vi "SMS Image Preview.vi"(7 "Calling VI Ref":refnum<vi>) -> ()   [LabVIEW 2021]
uses:
  <vilib>/Utility/miscctls.llb/LVPointTypeDef.ctl
  Hardware Configuration/Hardware Configuration Controls/Device Function.ctl
  SMS Image Preview Type Defs/SMS Image Preview Notifier Type.ctl
  SMS Image Preview Type Defs/SMS Image Preview Actions.ctl
  <vilib>/vision/Image Controls.llb/IMAQ Image.ctl
  Device Library/Cameras/Hamamatsu/Orca Flash/Orca Flash Controls/Orca Flash Actions.ctl
  Hardware Configuration/Hardware Configuration Controls/Device Type.ctl
  Device Library/FPGA/FPGA Controls/FPGA Action.ctl
  Device Library/Cameras/Camera Controls/Camera IMAQ Key Info.ctl
  Device Library/Lasers/Laser Controls/Laser Actions.ctl
  Device Library/Lasers/Laser Controls/Laser Settings.ctl
  Device Library/Lasers/Laser Controls/Laser Parameters.ctl
  <vilib>/Analysis/baseanly.llb/Mean (DBL).vi
  <vilib>/vision/NI_Vision_Development_Module.lvlib
  <vilib>/Analysis/NI_AALBase.lvlib
panel:
  in  "Laser":u16(ring) items=["405", "488"]
  in  "YOffset":i32=-1
  in  "XOffset":i32=1
  in  "Angle (degrees)":sgl format="%.2f"
  out "Current Emitter No.":u16
  in  "Duration":u32 max=65535 step=1
  in  "P Const.":dbl=0.5
  in  "Target Emitter No.":u16=3
  in  "Lock Density":bool
  in  "Average Frame No.":i32=2
  in  "Edge Size":i32=12
  in  "Use Quadrant":bool
  in  "Reset Plot":bool
  out "Blink No. vs. Time":cluster{dbl[], u16[]}(graph)
  in  "Accumulate":bool
  in  "Blink Sensitivity":sgl=10.0
  in  "Image Display":bool
  in  "SMS Preview":bool
  in  "Camera ROI":bool
  in  "Camera":i32(ring) items=["Hamamatsu-Camera-Primary-0"]
  in  "Quit":bool
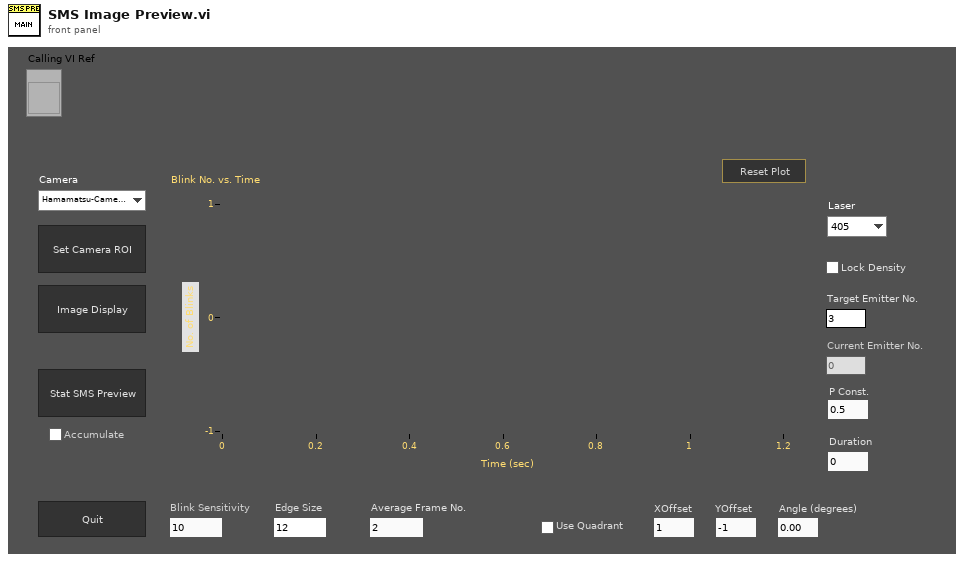
[diagram p1: front panel]
types:
  T1 = typedef "Device Function.ctl" = enum16{"Primary", "Secondary", "Overview", "Wide Field Drift Correction", "642 nm Excitation", "560 nm Excitation", "940 nm Excitation", "546 nm Excitation", "488 nm Excitation", "405 nm Excitation", "Objective Drift Correction", "4Pi Focus Lock", "4Pi Objective Lock", "Objective XY", "Objective Z", "Sample XY", "Sample Coarse Z", "Sample Z", "4Pi Lower", "4Pi Upper", "Em Small", "Em Large", "Ex Small", "Ex Large", "Mojo", "Adj Cavity", "Line Scanning", "Alert"}
  T2 = typedef "Image Type" = u32
  T3 = typedef "FPGA Action.ctl" = enum16{"Set Laser Mode", "Set Sequence", "Set Duration", "Write Check", "Idle", "Quit"}
  T4 = typedef "Device Type.ctl" = enum16{"AOTF", "Camera", "Deformable Mirror", "Laser", "Flip Mirror", "Shutter", "Stage", "Waveform", "FPGA", "Filter Wheel", "Email"}
  T5 = enum8{"Enabled", "Disabled", "Disabled and Grayed Out"}
  T6 = typedef "Orca Flash Actions.ctl" = enum16{"IDLE", "PREVIEW", "RECORD", "Send Trigger", "SOFT TRIGGER", "Record Settings", "SETPARAM", "GETPARAM", "SETROI", "GETROI", "PROGRESSIVE MODE", "AREA MODE", "STATUS", "QUIT"}
  T7 = typedef "SMS Image Preview Actions.ctl" = enum16{"Idle", "Start SMS Preview", "Get Image", "Get Quad", "Sum Quad", "Convolve and Threshold", "Subtract > Dilate", "And Image", "Remove Edge", "Update Plot", "Update Duration", "Abort", "Exit Loop", "Quit"}
  T8 = typedef "SMS Image Preview Notifier Type.ctl" = cluster{"Action":T7, "Camera Notifier Name":string, "Camera Image (U16)":T9, "Camera ROI":cluster{"Global Rectangle":i32[], "Contours":cluster{"Contour Type":u32, "ROI Type":u32, "Points":i32[]}[]}, "SMS Preview (U16)":T9, "Camera ROI (U16)":T9, "Threshold (U16)":T9, "Subtracted > Dilated (U16)":T9, "And Image (U16)":T9, "Camera ROI (SGL)":T9, "Conv 5 x 5 (SGL)":T9, "Conv 11 x 11 (SGL)":T9, "Subtracted (SGL)":T9, "Dilated (SGL)":T9, "Subtracted > Dilated (SGL)":T9, "Ones 5 x 5":sgl[][], "Ones 11 x 11":sgl[][], "Ones 7 x 7":i32[][], "Quads":T9[], "Edge Removed (U16)":T9, "Laser Notifier Name":string, "FPGA Notifier Name":string, "Duration":u32, "Quad 3 TM":T9}
  T9 = typedef "IMAQ Image.ctl" = refnum<image>
  T10 = enum16{"Always On", "Always Off", "Off While Running"}
  T11 = typedef "LVPointTypeDef.ctl" = cluster{"Horizontal":i16, "Vertical":i16}
  T12 = typedef "Camera IMAQ Key Info.ctl" = cluster{"Frame":u32, "Sensor Height":i32, "Sensor Width":i32, "ROI Height":i32, "ROI Width":i32, "ROI Enable?":bool, "Bit per Pixel":u8}
  T13 = enum32{"Average", "Min", "Max", "Clear  if < ", "Clear  if < or =", "Clear  if =", "Clear  if > or =", "Clear  if >"}
  T14 = enum32{"AutoM", "Close", "Dilate", "Erode", "Gradient", "Gradient in", "Gradient out", "HitMiss", "Open", "PClose", "POpen", "Thick", "Thin"}
  T15 = enum32{"Invalid", "Standard", "Closed", "Hidden", "Minimized", "Maximized"}
  T16 = cluster{"Global Rectangle":i32[], "Contours":cluster{"Contour Type":u32, "ROI Type":u32, "Points":i32[]}[]}
  T17 = typedef "Laser Parameters.ctl" = enum16{"Wavelength (nm)", "Pulsing?", "Rep. Rate", "External Control", "Enable Fine", "Fine A", "Fine B", "Channel No."}
  T18 = typedef "Laser Settings.ctl" = cluster{"Laser Parameters":T17, "Value":dbl}
  T19 = typedef "Laser Actions.ctl" = enum16{"Error Check", "Set On/Off", "Set Power", "Set Parameter", "Get Power", "Get Status", "Get Parameter", "Quit"}
  T20 = cluster{"histogram":u32[], "Minimal Value":sgl, "Maximal Value":sgl, "Starting Value":sgl, "Interval Width":sgl, "Mean Value":sgl, "Standard  Variation":sgl, "Area (pixels)":i32}
  T21 = typedef "LVRectTypeDef.ctl" = cluster{"Left":i16, "Top":i16, "Right":i16, "Bottom":i16}
  T22 = typedef "LVBoundsTypeDef.ctl" = cluster{"Width":u32, "Height":u32}
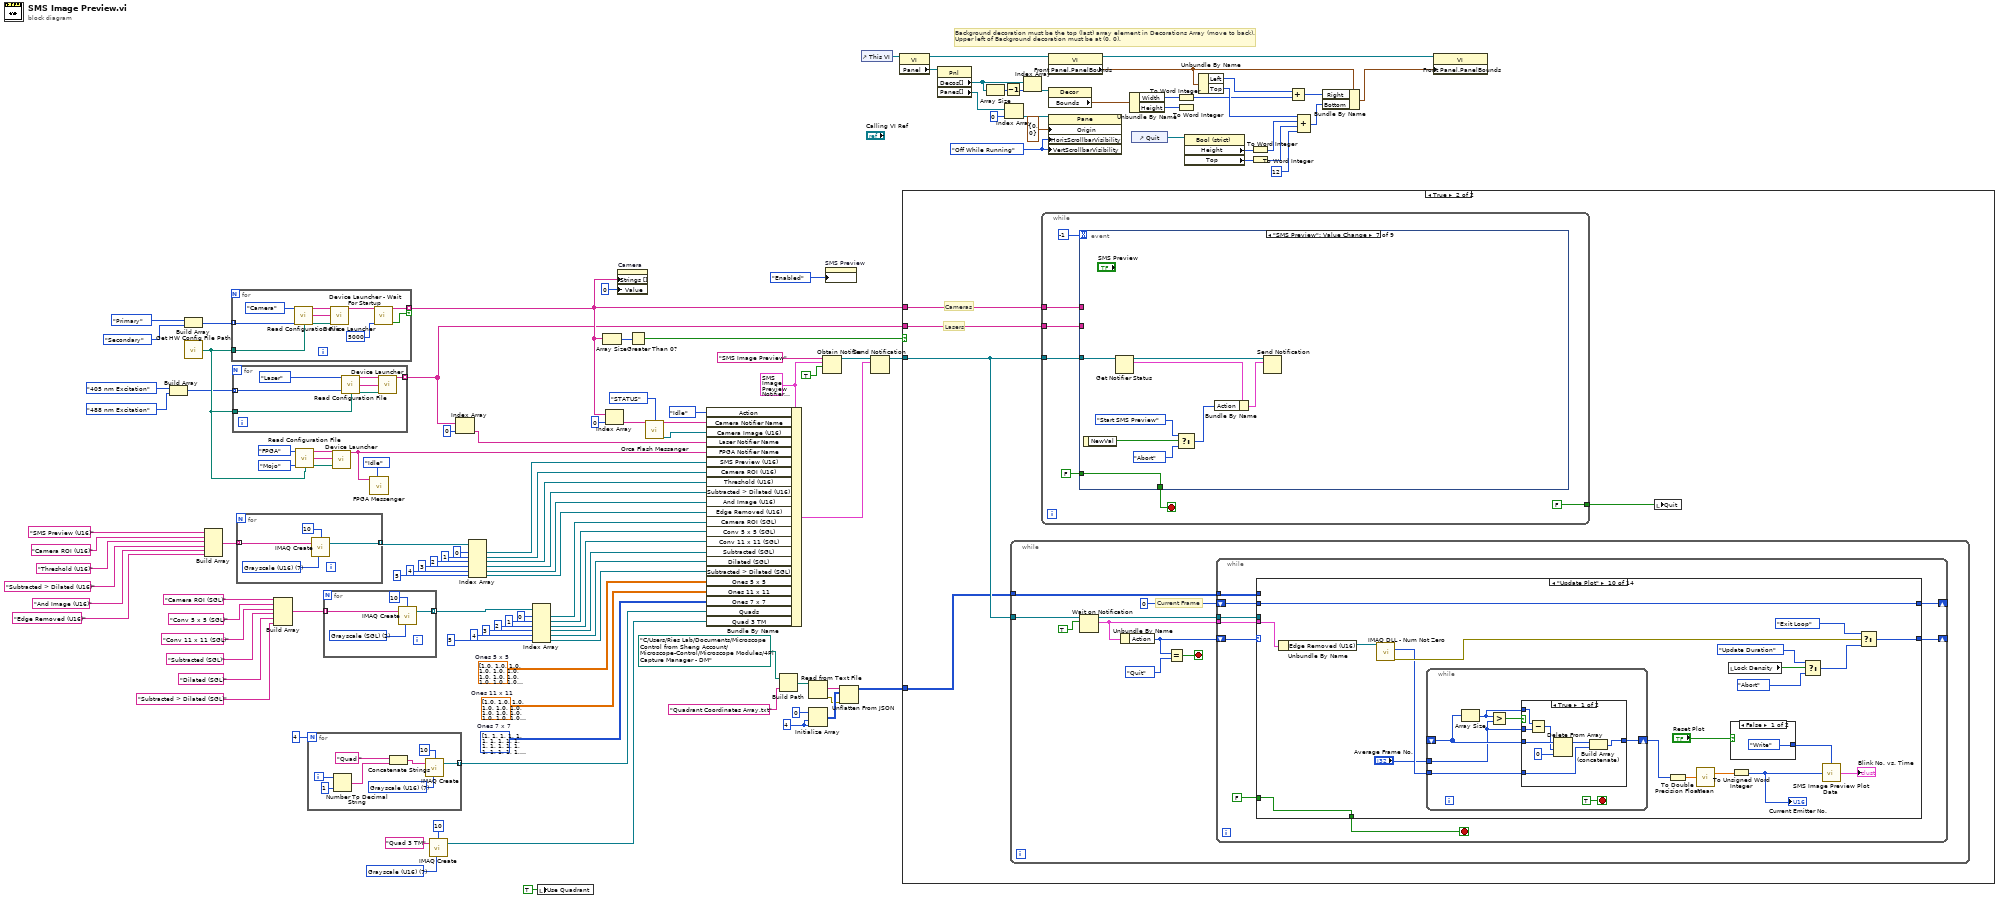
[diagram p0: block diagram]
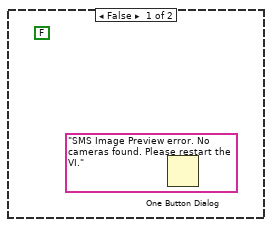
[diagram p2: hidden frame]
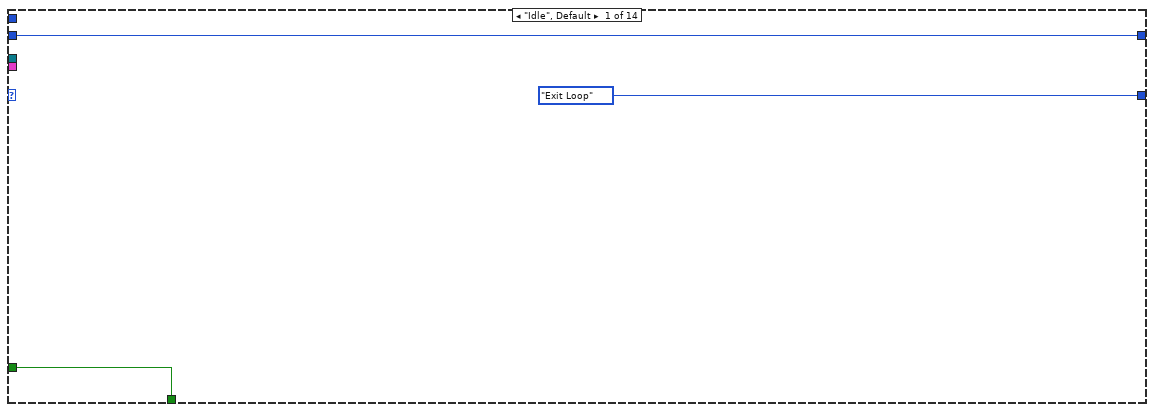
[diagram p3: hidden frame]
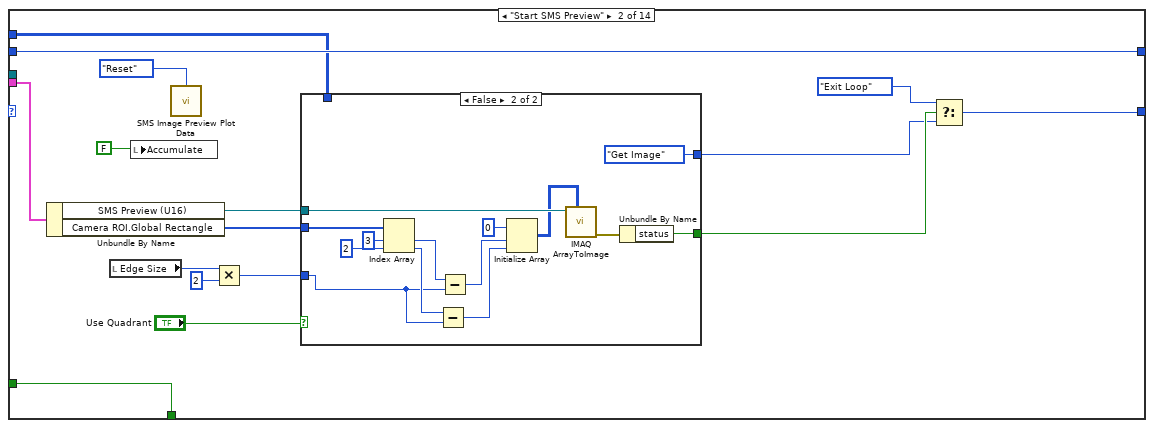
[diagram p4: hidden frame]
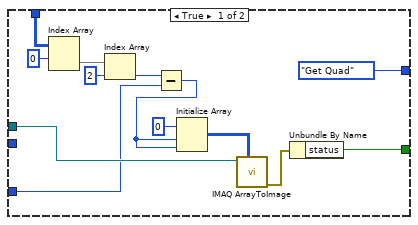
[diagram p5: hidden frame]
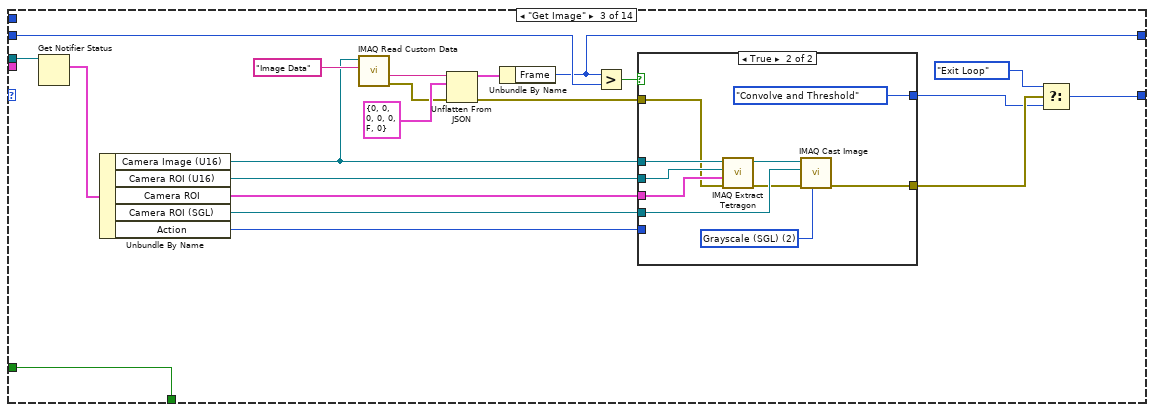
[diagram p6: hidden frame]
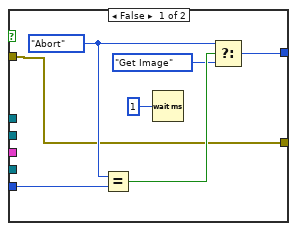
[diagram p7: hidden frame]
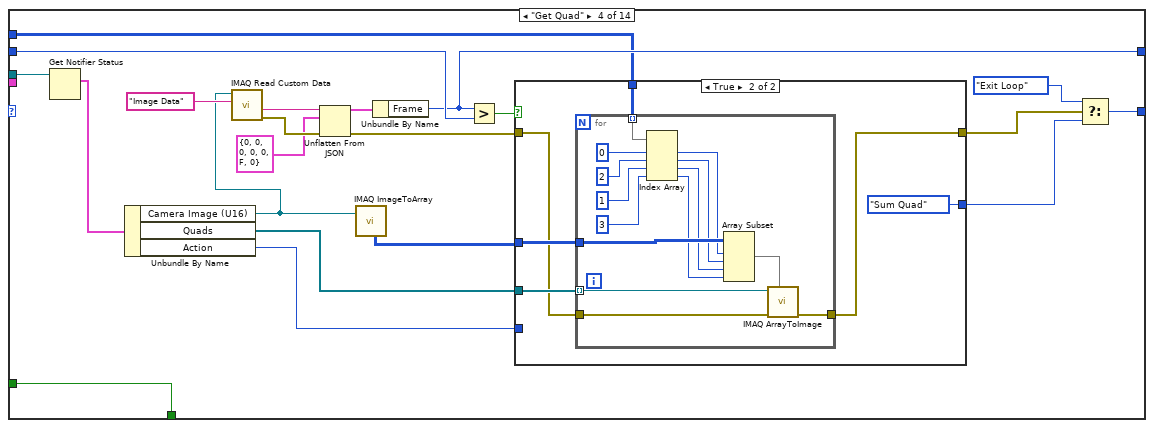
[diagram p8: hidden frame]
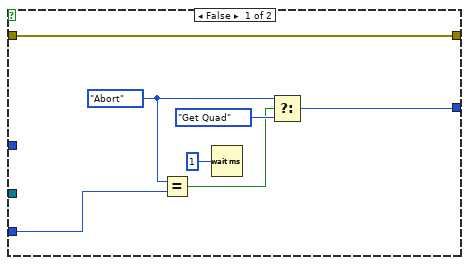
[diagram p9: hidden frame]
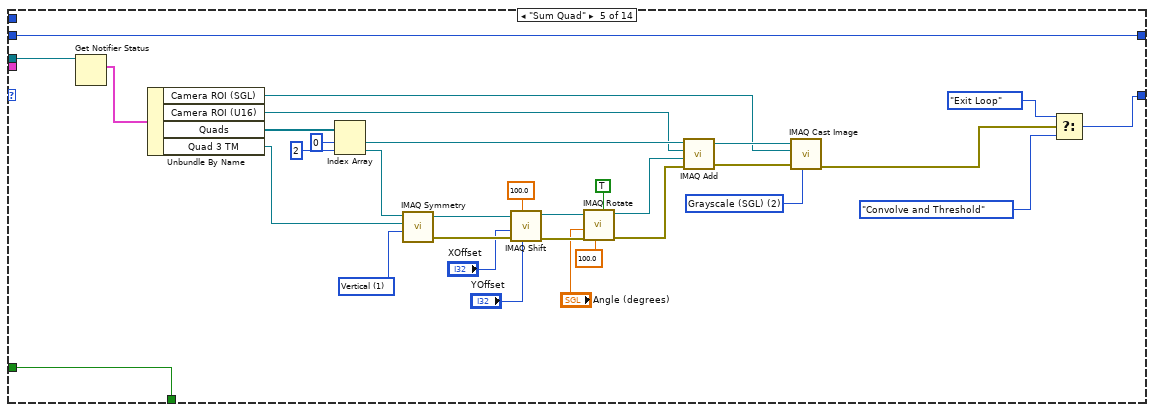
[diagram p10: hidden frame]
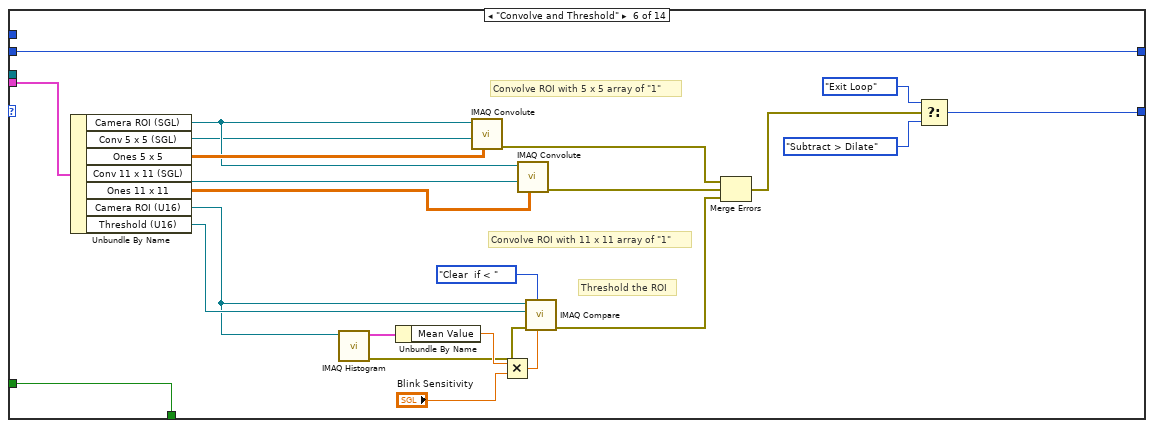
[diagram p11: hidden frame]
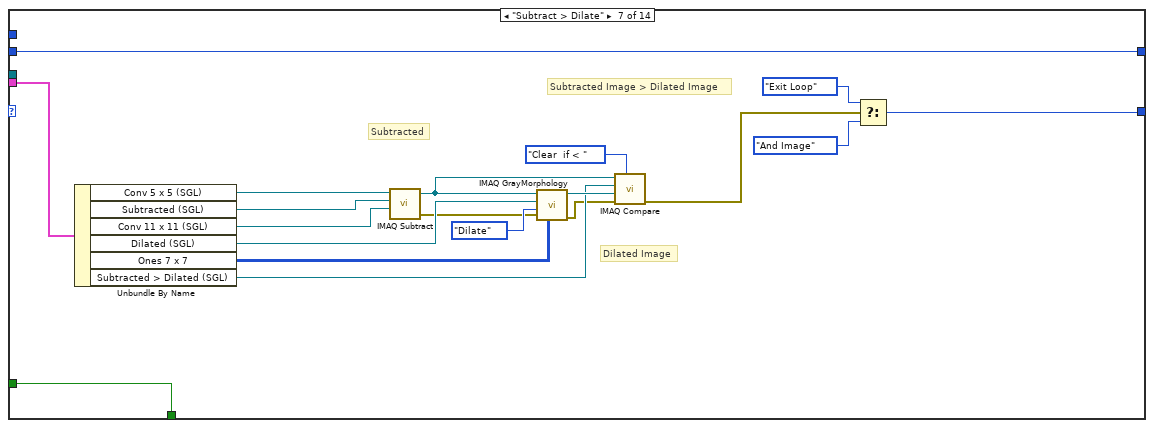
[diagram p12: hidden frame]
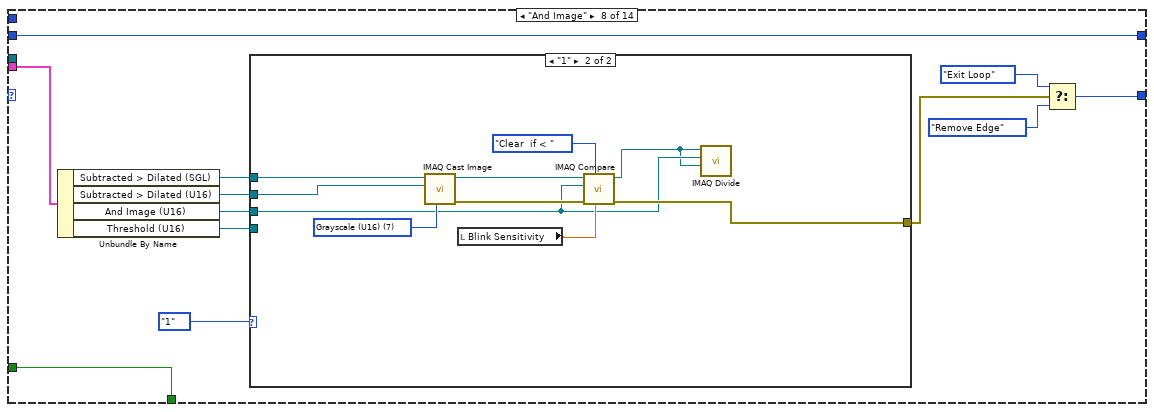
[diagram p13: hidden frame]
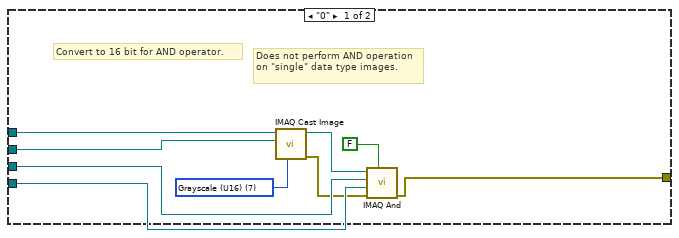
[diagram p14: hidden frame]
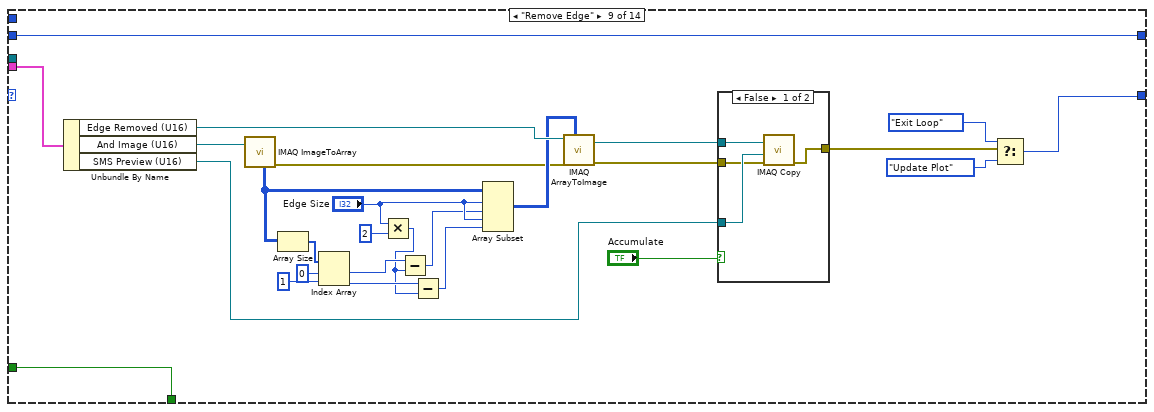
[diagram p15: hidden frame]
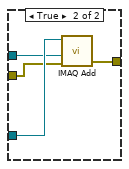
[diagram p16: hidden frame]
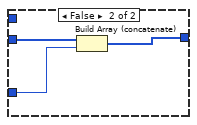
[diagram p17: hidden frame]
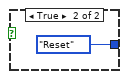
[diagram p18: hidden frame]
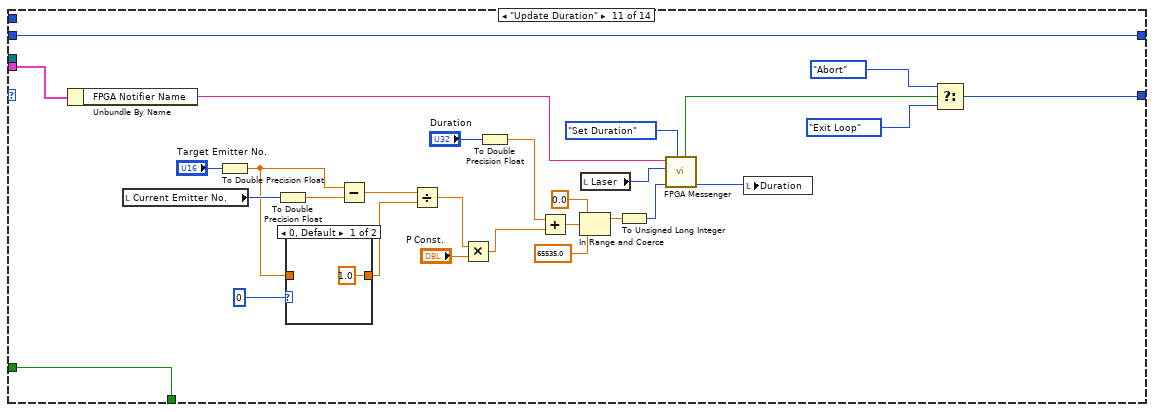
[diagram p19: hidden frame]
diagram:
  w12 = T2 7 items=["Grayscale (U8)", "Grayscale (I16)", "Grayscale (SGL)", "Complex (CSG)", "RGB (U32)", "HSL (U32)", "RGB (U64)", "Grayscale (U16)"] ("Image Type")
  w27 = 4 ("dimension size")
  w38 = i32[][] [[1, 1, 1, 1, 1, 1, 1], [1, 1, 1, 1, 1, 1, 1], [1, 1, 1, 1, 1, 1, 1], [1, 1, 1, 1, 1, 1, 1], [1, 1, 1, 1, 1, 1, 1], [1, 1, 1, 1, 1, 1, 1], [1, 1, 1, 1, 1, 1, 1]]  # Ones 7 x 7
  w39 = sgl[][] [[1.0, 1.0, 1.0, 1.0, 1.0, 1.0, 1.0, 1.0, 1.0, 1.0, 1.0], [1.0, 1.0, 1.0, 1.0, 1.0, 1.0, 1.0, 1.0, 1.0, 1.0, 1.0], [1.0, 1.0, 1.0, 1.0, 1.0, 1.0, 1.0, 1.0, 1.0, 1.0, 1.0], [1.0, 1.0, 1.0, 1.0, 1.0, 1.0, 1.0, 1.0, 1.0, 1.0, 1.0], [1.0, 1.0, 1.0, 1.0, 1.0, 1.0, 1.0, 1.0, 1.0, 1.0, 1.0], [1.0, 1.0, 1.0, 1.0, 1.0, 1.0, 1.0, 1.0, 1.0, 1.0, 1.0], [1.0, 1.0, 1.0, 1.0, 1.0, 1.0, 1.0, 1.0, 1.0, 1.0, 1.0], [1.0, 1.0, 1.0, 1.0, 1.0, 1.0, 1.0, 1.0, 1.0, 1.0, 1.0], [1.0, 1.0, 1.0, 1.0, 1.0, 1.0, 1.0, 1.0, 1.0, 1.0, 1.0], [1.0, 1.0, 1.0, 1.0, 1.0, 1.0, 1.0, 1.0, 1.0, 1.0, 1.0], [1.0, 1.0, 1.0, 1.0, 1.0, 1.0, 1.0, 1.0, 1.0, 1.0, 1.0]]  # Ones 11 x 11
  w40 = sgl[][] [[1.0, 1.0, 1.0, 1.0, 1.0], [1.0, 1.0, 1.0, 1.0, 1.0], [1.0, 1.0, 1.0, 1.0, 1.0], [1.0, 1.0, 1.0, 1.0, 1.0], [1.0, 1.0, 1.0, 1.0, 1.0]]  # Ones 5 x 5
  w35 = T8 {"Action"=enum."Idle", "Camera Notifier Name"="", "Camera Image (U16)"=refnum, "Camera ROI"={"Global Rectangle"=[], "Contours"=[]}, "SMS Preview (U16)"=refnum, "Camera ROI (U16)"=refnum, "Threshold (U16)"=refnum, "Subtracted > Dilated (U16)"=refnum, "And Image (U16)"=refnum, "Camera ROI (SGL)"=refnum, "Conv 5 x 5 (SGL)"=refnum, "Conv 11 x 11 (SGL)"=refnum, "Subtracted (SGL)"=refnum, "Dilated (SGL)"=refnum, "Subtracted > Dilated (SGL)"=refnum, "Ones 5 x 5"=[], "Ones 11 x 11"=[], "Ones 7 x 7"=[], "Quads"=[], "Edge Removed (U16)"=refnum, "Laser Notifier Name"="", "FPGA Notifier Name"="", "Duration"=0, "Quad 3 TM"=refnum} ("SMS Image Preview Notifier Type")
  w105 = T10."Off While Running" ("Vertical Scrollbar Visibility")
  # "Background decoration must be the top (last) array element in Decorations Array (move to back).\nUpper left of Background decoration must be at (0, 0)."
  n1 = Build Array(Device_Function."405 nm Excitation" ("Device Function"), Device_Function."488 nm Excitation" ("Device Function")) -> (w5:T1[])
  n2 = Build Array(Device_Function."Primary" ("Device Function"), Device_Function."Secondary" ("Device Function")) -> (w91:T1[])
  n3 = call "Get HW Config File Path.vi"() -> ("File Path"=w15:path)  [unwired: 14 in, 1 out]
  n4 = Build Array("SMS Preview (U16)" ("Image Name"), "Camera ROI (U16)" ("Image Name"), "Threshold (U16)" ("Image Name"), "Subtracted > Dilated (U16)" ("Image Name"), "And Image (U16)" ("Image Name"), "Edge Removed (U16)" ("element")) -> (w50:string[])
  n5 = for {
    tunnel: w91 -> [w128] mode=indexing
    tunnel: w15 -> [w127]
    tunnel: [w125] -> w81 mode=indexing if=w124
    n6 = call "Read Configuration File.vi"("Device Type"=Device_Type."Camera", "Device Function"=w128, "Config File Path"=w127) -> ("Unique Notifier Name"=w130:string, "Device Ports/IDs/Channels"=w132:string[], "Device Engine Path"=w131:path)  [unwired: 9 in, 1 out]
    n7 = call "Device Launcher.vi"("Notifier Name"=w130, "Device Ports/IDs/Channels"=w132, "Device Engine Path"=w131) -> ("Notifier Name"=w126:string)  [unwired: 11 in, 1 out]
    n8 = call "Device Launcher - Wait For Startup.vi"("Notifier Name"=w126, "Wait Time (ms)"=5000) -> ("Notifier Name (Dup)"=w125:string, "Running?"=w124:bool)  [unwired: 12 in]
  }
  n9 = for {
    tunnel: [w135] -> w2 mode=indexing
    tunnel: w15 -> [w134]
    tunnel: w5 -> [w133] mode=indexing
    n10 = call "Read Configuration File.vi"("Device Type"=Device_Type."Laser", "Device Function"=w133, "Config File Path"=w134) -> ("Unique Notifier Name"=w138:string, "Device Ports/IDs/Channels"=w137:string[], "Device Engine Path"=w136:path)  [unwired: 9 in, 1 out]
    n11 = call "Device Launcher.vi"("Notifier Name"=w138, "Device Ports/IDs/Channels"=w137, "Device Engine Path"=w136) -> ("Notifier Name"=w135:string)  [unwired: 11 in, 1 out]
  }
  n12 = for {
    tunnel: w50 -> [w141] mode=indexing
    tunnel: [w140] -> w51 mode=indexing
    w142 = T2 7 items=["Grayscale (U8)", "Grayscale (I16)", "Grayscale (SGL)", "Complex (CSG)", "RGB (U32)", "HSL (U32)", "RGB (U64)", "Grayscale (U16)"] ("Image Type")
    n13 = call "IMAQ Create"("Border Size"=10, "Image Name"=w141, "Image Type"=w142) -> ("New Image"=w140:T9)  [unwired: 2 in, 1 out]
  }
  n14 = Build Array("Camera ROI (SGL)" ("Image Name"), "Conv 5 x 5 (SGL)" ("Image Name"), "Conv 11 x 11 (SGL)" ("Image Name"), "Subtracted (SGL)" ("Image Name"), "Dilated (SGL)" ("Image Name"), "Subtracted > Dilated (SGL)" ("Image Name")) -> (w70:string[])
  n15 = call "Read Configuration File.vi"("Device Type"=Device_Type."FPGA", "Device Function"=Device_Function."Mojo", "Config File Path"=w15) -> ("Unique Notifier Name"=w18:string, "Device Ports/IDs/Channels"=w17:string[], "Device Engine Path"=w16:path)  [unwired: 9 in, 1 out]
  n16 = for {
    N: 4 -> [_]
    tunnel: [w149] -> w34 mode=indexing
    i -> [w148]
    w151 = T2 7 items=["Grayscale (U8)", "Grayscale (I16)", "Grayscale (SGL)", "Complex (CSG)", "RGB (U32)", "HSL (U32)", "RGB (U64)", "Grayscale (U16)"] ("Image Type")
    n17 = Number To Decimal String(number=w148, width (-)=i16 1) -> (decimal integer string=w145:string)
    n18 = Concatenate Strings("Quad " ("Image Name"), w145) -> (w144:string)
    n19 = call "IMAQ Create"("Border Size"=10, "Image Name"=w144, "Image Type"=w151) -> ("New Image"=w149:T9)  [unwired: 2 in, 1 out]
  }
  n20 = for {
    tunnel: w70 -> [w153] mode=indexing
    tunnel: [w152] -> w69 mode=indexing
    w154 = T2 2 items=["Grayscale (U8)", "Grayscale (I16)", "Grayscale (SGL)", "Complex (CSG)", "RGB (U32)", "HSL (U32)", "RGB (U64)", "Grayscale (U16)"] ("Image Type")
    n21 = call "IMAQ Create"("Border Size"=10, "Image Name"=w153, "Image Type"=w154) -> ("New Image"=w152:T9)  [unwired: 2 in, 1 out]
  }
  n22 = call "Device Launcher.vi"("Notifier Name"=w18, "Device Ports/IDs/Channels"=w17, "Device Engine Path"=w16) -> ("Notifier Name"=w14:string)  [unwired: 11 in, 1 out]
  n23 = call "FPGA Messenger.vi"("FPGA Action"=FPGA_Action."Idle", "Notifier Name"=w14) -> ()  [unwired: 4 in, 6 out]
  n24 = call "IMAQ Create"("Border Size"=10, "Image Name"="Quad 3 TM", "Image Type"=w12) -> ("New Image"=w9:T9)  [unwired: 2 in, 1 out]
  n25 = Index Array(array=w2, index=0) -> (element=w3:string)
  n26 = Index Array(array=w51, index #1=0 ("index"), index #2=1 ("index"), index #3=2 ("index"), index #4=3 ("index"), index #5=4 ("index"), index #6=5 ("index")) -> (element #1=w49:T9, element #2=w48:T9, element #3=w47:T9, element #4=w23:T9, element #5=w22:T9, element #6=w21:T9)
  n27 = Index Array(array=w69, index #1=0 ("index"), index #2=1 ("index"), index #3=2 ("index"), index #4=3 ("index"), index #5=4 ("index"), index #6=5 ("index")) -> (element #1=w46:T9, element #2=w45:T9, element #3=w44:T9, element #4=w43:T9, element #5=w42:T9, element #6=w41:T9)
  n28 = local write "Use Quadrant"(TRUE ("Use Quadrant")) -> ()
  n29 = Array Size(array=w81) -> (size(s)=w90:i32)
  n30 = Index Array(array=w81, index=0) -> (element=w79:string)
  n31 = property on="Camera" class="Ring (strict)"("Strings []"=w81, "Value"=0) -> ()  [unwired: 2 in, 2 out]
  n32 = Greater Than 0?(x=w90) -> (x > 0?=w89:bool)
  n33 = call "Orca Flash Messanger.vi"("Notifier Name"=w79, "Camera Actions"=Orca_Flash_Actions."STATUS") -> ("Notifier Name Dup"=w78:string, "Image Ref"=w76:T9)  [unwired: 9 in, 3 out]
  n34 = Bundle By Name(cluster=w35, "Action"=SMS_Image_Preview_Actions."Idle", "Camera Notifier Name"=w78, "Camera Image (U16)"=w76, "Laser Notifier Name"=w3, "FPGA Notifier Name"=w14, "SMS Preview (U16)"=w49, "Camera ROI (U16)"=w48, "Threshold (U16)"=w47, "Subtracted > Dilated (U16)"=w23, "And Image (U16)"=w22, "Edge Removed (U16)"=w21, "Camera ROI (SGL)"=w46, "Conv 5 x 5 (SGL)"=w45, "Conv 11 x 11 (SGL)"=w44, "Subtracted (SGL)"=w43, "Dilated (SGL)"=w42, "Subtracted > Dilated (SGL)"=w41, "Ones 5 x 5"=w40, "Ones 11 x 11"=w39, "Ones 7 x 7"=w38, "Quads"=w34, "Quad 3 TM"=w9) -> (w82:T8)
  n35 = Build Path(base path=path "C:/Users/Ries Lab/Documents/Microscope Control from Sheng Account/Microscope-Control/Microscope Modules/4Pi Capture Manager - DM" ("path"), name or relative path="Quadrant Coordinates Array.txt") -> (appended path=w30:path)
  n36 = Read from Text File(file (use dialog)=w30) -> (text=w29:string, error out=w28:errorcluster)  [unwired: 3 in, 2 out]
  n37 = Initialize Array(0 ("element"), w27, w27) -> (w31:i32[][])
  n38 = Obtain Notifier(name (unnamed)="SMS Image Preview", notification data type=w35, create if not found? (T)=TRUE) -> (notifier out=w85:refnum<notifier>)  [unwired: 1 in, 2 out]
  n39 = property on="SMS Preview" class="Bool (strict)"("DisabledEnum"=T5."Enabled" ("Disabled")) -> ()  [unwired: 2 in, 2 out]
  n40 = Unflatten From JSON(JSON string=w29, type and defaults=w31, error in (no error)=w28) -> (value=w26:i32[][])  [unwired: 4 in, 1 out]
  n41 = control-ref of="This VI"() -> (w97:refnum<vi>)
  n42 = Send Notification(notification=w82, notifier=w85) -> (notifier out=w83:refnum<notifier>)  [unwired: 1 in, 1 out]
  n43 = property class="VI"(reference=w97) -> (reference out=w106:refnum<vi>, "Panel"=w98:refnum<vi>)  [unwired: 1 in, 1 out]
  n44 = case shown="True" w89 {
    tunnel: w81 -> [_ w161]
    tunnel: w83 -> [_ w159]
    tunnel: w26 -> [_ w158]
    tunnel: w2 -> [_ w157]
    frame False {
      (unwired) FALSE
      n45 = One Button Dialog(message="SMS Image Preview error. No cameras found. Please restart the VI.") -> ()  [unwired: 1 in, 1 out]
    }
    frame True {
      # "Lasers"
      # "Cameras"
      n46 = while {
        tunnel: w159 -> [w170]
        tunnel: w158 -> [w162]
        stop <- w167 stop-if-true
        # "Current Frame"
        n47 = Wait on Notification(notifier=w170, ignore previous (F)=TRUE) -> (notifier out=w163:refnum<notifier>, notification=w165:T8)  [unwired: 2 in, 2 out]
        n48 = Unbundle By Name(w165) -> ("Action"=w166:T7)
        n49 = Equal?(x=w166, y=SMS_Image_Preview_Actions."Quit") -> (x = y?=w167:bool)
        n50 = while {
          shift-right: [w171] -> _
          shift-left: w166 -> [w179]
          tunnel: w165 -> [w178]
          shift-right: [w176] -> _
          shift-left: u32 0 -> [w177]
          tunnel: w163 -> [w175]
          tunnel: w162 -> [w172]
          stop <- w173 stop-if-true
          n51 = case shown="\"Update Plot\"" w179 {
            tunnel: w178 -> [_ w196 _ _ _ w365 w384 w396 w432 w467 w508 _ _ _]
            tunnel: [SMS_Image_Preview_Actions."Exit Loop" ("y") w193 w228 w266 w321 w346 w367 w387 w424 w469 w510 w526 SMS_Image_Preview_Actions."Exit Loop" ("f") SMS_Image_Preview_Actions."Quit" ("f")] -> w171
            tunnel: w177 -> [w181 w198 w242 w275 w332 w366 w385 w397 w427 w470 w514 w531 w537 w554]
            tunnel: [w181 w198 w241 w274 w332 w366 w385 w397 w427 w470 w514 w531 w537 w554] -> w176
            tunnel: w175 -> [_ _ w236 w283 w333 _ _ _ _ _ _ w530 _ w551]
            tunnel: FALSE -> [w180 w197 w237 w284 w320 w356 w373 w391 w423 w462 w509 w524 _ _]
            tunnel: [w180 w197 w237 w284 w320 w356 w373 w391 w423 w462 w509 w524 TRUE TRUE] -> w173
            tunnel: w172 -> [_ w187 _ w265 _ _ _ _ _ _ _ _ _ _]
            frame "Idle", Default {
            }
            frame "Start SMS Preview" {
              n52 = Unbundle By Name(w196) -> ("SMS Preview (U16)"=w194:T9, "Camera ROI.Global Rectangle"=w195:i32[])
              n53 = local read "Edge Size"() -> (w185:i32)
              n54 = local write "Accumulate"(FALSE ("Accumulate")) -> ()
              n55 = call "SMS Image Preview Plot Data.vi"("Plot Data Actions"=enum16{"Read", "Write", "Reset"}."Reset") -> ()  [unwired: 14 in, 1 out]
              n56 = Multiply(x=w185, y=2) -> (x*y=w183:i32)
              n57 = case shown="False" "Use Quadrant" {
                tunnel: w195 -> [_ w225]
                tunnel: w194 -> [w202 w221]
                tunnel: [w208 w218] -> w192
                tunnel: [SMS_Image_Preview_Actions."Get Quad" ("y") SMS_Image_Preview_Actions."Get Image" ("y")] -> w188
                tunnel: w187 -> [w206 _]
                tunnel: w183 -> [w200 w213]
                frame True {
                  n58 = Index Array(array=w206, index (row)=0) -> (element=w204:i32[])  [unwired: 1 in]
                  n59 = Index Array(array=w204, index=2) -> (element=w201:i32)
                  n60 = Subtract(x=w201, y=w200) -> (x-y=w199:i32)
                  n61 = Initialize Array(u16 0 ("index"), w199, w199) -> (w210:u16[][])
                  n62 = call "IMAQ ArrayToImage"("Image Pixels (U16)"=w210, "Image"=w202) -> ("error out"=w211:errorcluster)  [unwired: 8 in, 1 out]
                  n63 = Unbundle By Name(w211) -> ("status"=w208:bool)
                }
                frame False {
                  n64 = Index Array(array=w225, index #1=3 ("index"), index #2=2 ("index")) -> (element #1=w216:i32, element #2=w214:i32)
                  n65 = Subtract(x=w214, y=w213) -> (x-y=w212:i32)
                  n66 = Subtract(x=w216, y=w213) -> (x-y=w215:i32)
                  n67 = Initialize Array(u16 0 ("index"), w215, w212) -> (w220:u16[][])
                  n68 = call "IMAQ ArrayToImage"("Image Pixels (U16)"=w220, "Image"=w221) -> ("error out"=w219:errorcluster)  [unwired: 8 in, 1 out]
                  n69 = Unbundle By Name(w219) -> ("status"=w218:bool)
                }
              }
              n70 = Select(t=SMS_Image_Preview_Actions."Exit Loop", s=w192, f=w188) -> (s? t:f=w193:T7)
            }
            frame "Get Image" {
              n71 = Get Notifier Status(notifier=w236) -> (current notification=w235:T8)  [unwired: 1 in, 4 out]
              n72 = Unbundle By Name(w235) -> ("Camera Image (U16)"=w239:T9, "Camera ROI (U16)"=w238:T9, "Camera ROI"=w226:T16, "Camera ROI (SGL)"=w233:T9, "Action"=w234:T7)
              n73 = call "IMAQ Read Custom Data"("Key"="Image Data", "Image"=w239) -> ("error out"=w232:errorcluster, "Custom Data Out"=w244:string)  [unwired: 7 in, 1 out]
              n74 = Unflatten From JSON(JSON string=w244, type and defaults=T12 {"Frame"=0, "Sensor Height"=0, "Sensor Width"=0, "ROI Height"=0, "ROI Width"=0, "ROI Enable?"=FALSE, "Bit per Pixel"=0} ("Camera IMAQ Key Info"), error in (no error)=w232) -> (value=w246:T12, error out=w231:errorcluster)  [unwired: 4 in]
              n75 = Unbundle By Name(w246) -> ("Frame"=w241:u32)
              n76 = Greater?(x=w241, y=w242) -> (0:w240:bool)
              n77 = case shown="True" w240 {
                tunnel: w239 -> [_ w263]
                tunnel: w238 -> [_ w262]
                tunnel: w226 -> [_ w261]
                tunnel: [w251 SMS_Image_Preview_Actions."Convolve and Threshold" ("y")] -> w229
                tunnel: w234 -> [w253 _]
                tunnel: w233 -> [_ w257]
                tunnel: w231 -> [w247 w256]
                tunnel: [w247 w254] -> w230
                frame False {
                  w252 = SMS_Image_Preview_Actions."Abort" ("x")
                  n78 = Equal?(x=w252, y=w253) -> (x = y?=w250:bool)
                  n79 = Wait (ms)(milliseconds to wait=u32 1) -> ()  [unwired: 1 out]
                  n80 = Select(t=w252, s=w250, f=SMS_Image_Preview_Actions."Get Image" ("y")) -> (s? t:f=w251:T7)
                }
                frame True {
                  w259 = T2 2 items=["Grayscale (U8)", "Grayscale (I16)", "Grayscale (SGL)", "Complex (CSG)", "RGB (U32)", "HSL (U32)", "RGB (U64)", "Grayscale (U16)"] ("Image Type")
                  n81 = call-poly "IMAQ Extract Tetragon"("error in (no error)"=w256, "ROI Descriptor"=w261, "Image Dst"=w262, "Image Src"=w263) -> ("error out"=w255:errorcluster, "Image Dst Out"=w258:T9)  [unwired: 6 in]
                  n82 = call "IMAQ Cast Image"("Image Type"=w259, "error in (no error)"=w255, "Image Dst"=w257, "Image Src"=w258) -> ("error out"=w254:errorcluster)  [unwired: 6 in, 1 out]
                }
              }
              n83 = Select(t=SMS_Image_Preview_Actions."Exit Loop", s=w230, f=w229) -> (s? t:f=w228:T7)
            }
            frame "Get Quad" {
              n84 = Get Notifier Status(notifier=w283) -> (current notification=w282:T8)  [unwired: 1 in, 4 out]
              n85 = Unbundle By Name(w282) -> ("Camera Image (U16)"=w267:T9, "Quads"=w281:T9[], "Action"=w272:T7)
              n86 = call "IMAQ Read Custom Data"("Key"="Image Data", "Image"=w267) -> ("error out"=w280:errorcluster, "Custom Data Out"=w278:string)  [unwired: 7 in, 1 out]
              n87 = Unflatten From JSON(JSON string=w278, type and defaults=T12 {"Frame"=0, "Sensor Height"=0, "Sensor Width"=0, "ROI Height"=0, "ROI Width"=0, "ROI Enable?"=FALSE, "Bit per Pixel"=0} ("Camera IMAQ Key Info"), error in (no error)=w280) -> (value=w276:T12, error out=w270:errorcluster)  [unwired: 4 in]
              n88 = call "IMAQ ImageToArray"("Image"=w267) -> ("Image Pixels (U16)"=w264:u16[][])  [unwired: 3 in, 4 out]
              n89 = Unbundle By Name(w276) -> ("Frame"=w274:u32)
              n90 = Greater?(x=w274, y=w275) -> (0:w273:bool)
              n91 = case shown="True" w273 {
                tunnel: w281 -> [_ w297]
                tunnel: w265 -> [_ w296]
                tunnel: w264 -> [_ w295]
                tunnel: w272 -> [w287 _]
                tunnel: [w286 w293] -> w269
                tunnel: w270 -> [w286 w294]
                tunnel: [w285 SMS_Image_Preview_Actions."Sum Quad" ("y")] -> w268
                frame False {
                  w288 = SMS_Image_Preview_Actions."Abort" ("x")
                  n92 = Equal?(x=w288, y=w287) -> (x = y?=w289:bool)
                  n93 = Wait (ms)(milliseconds to wait=u32 1) -> ()  [unwired: 1 out]
                  n94 = Select(t=w288, s=w289, f=SMS_Image_Preview_Actions."Get Quad" ("y")) -> (s? t:f=w285:T7)
                }
                frame True {
                  n95 = for {
                    tunnel: w297 -> [w310] mode=indexing
                    tunnel: w295 -> [w311]
                    tunnel: w296 -> [w308] mode=indexing
                    tunnel: w294 -> [w299]
                    tunnel: [w298] -> w293
                    n96 = Index Array(array=w308, index #1=0 ("index"), index #2=2 ("index"), index #3=1 ("index"), index #4=3 ("index")) -> (element #1=w306:i32, element #2=w305:i32, element #3=w301:i32, element #4=w300:i32)
                    n97 = Array Subset(array=w311, index (row)=w306, length (row)=w305, index (col)=w301, length (col)=w300) -> (w309:u16[][])
                    n98 = call "IMAQ ArrayToImage"("Image Pixels (U16)"=w309, "error in (no error)"=w299, "Image"=w310) -> ("error out"=w298:errorcluster)  [unwired: 7 in, 1 out]
                  }
                }
              }
              n99 = Select(t=SMS_Image_Preview_Actions."Exit Loop", s=w269, f=w268) -> (s? t:f=w266:T7)
            }
            frame "Sum Quad" {
              w318 = u32 1 items=["Horizontal", "Vertical", "Central", "1st Diagonal", "2nd Diagonal"] ("Type of Symmetry")
              w326 = T2 2 items=["Grayscale (U8)", "Grayscale (I16)", "Grayscale (SGL)", "Complex (CSG)", "RGB (U32)", "HSL (U32)", "RGB (U64)", "Grayscale (U16)"] ("Image Type")
              n100 = Get Notifier Status(notifier=w333) -> (current notification=w331:T8)  [unwired: 1 in, 4 out]
              n101 = Unbundle By Name(w331) -> ("Camera ROI (SGL)"=w325:T9, "Camera ROI (U16)"=w329:T9, "Quads"=w330:T9[], "Quad 3 TM"=w312:T9)
              n102 = Index Array(array=w330, index #1=0 ("index"), index #2=2 ("index")) -> (element #1=w336:T9, element #2=w319:T9)
              n103 = call "IMAQ Symmetry"("Type of Symmetry"=w318, "Image Dst"=w312, "Image Src"=w319) -> ("error out"=w317:errorcluster, "Image Dst Out"=w316:T9)  [unwired: 2 in]
              n104 = call "IMAQ Shift"("YOffset"="YOffset", "Replace Value"=sgl 100.0, "error in (no error)"=w317, "XOffset"="XOffset", "Image Src"=w316) -> ("error out"=w335:errorcluster, "Image Dst Out"=w340:T9)  [unwired: 5 in]
              n105 = call "IMAQ Rotate"("Maintain Size"=TRUE, "Replace Value"=sgl 100.0, "error in (no error)"=w335, "Angle (degrees)"="Angle (degrees)", "Image Src"=w340) -> ("error out"=w334:errorcluster, "Image Dst Out"=w337:T9)  [unwired: 5 in]
              n106 = call "IMAQ Add"("Image Src A"=w336, "Image Dst"=w329, "Image Src B"=w337, "error in (no error)"=w334) -> ("Image Dst Out"=w328:T9, "error out"=w327:errorcluster)  [unwired: 3 in]
              n107 = call "IMAQ Cast Image"("Image Type"=w326, "error in (no error)"=w327, "Image Dst"=w325, "Image Src"=w328) -> ("error out"=w322:errorcluster)  [unwired: 6 in, 1 out]
              n108 = Select(t=SMS_Image_Preview_Actions."Exit Loop", s=w322, f=SMS_Image_Preview_Actions."Convolve and Threshold") -> (s? t:f=w321:T7)
            }
            frame "Convolve and Threshold" {
              # "Threshold the ROI"
              # "Convolve ROI with 11 x 11 array of \"1\""
              # "Convolve ROI with 5 x 5 array of \"1\""
              n109 = Unbundle By Name(w365) -> ("Camera ROI (SGL)"=w358:T9, "Conv 5 x 5 (SGL)"=w355:T9, "Ones 5 x 5"=w364:sgl[][], "Conv 11 x 11 (SGL)"=w354:T9, "Ones 11 x 11"=w363:sgl[][], "Camera ROI (U16)"=w353:T9, "Threshold (U16)"=w357:T9)
              n110 = call "IMAQ Histogram"("Image"=w353) -> ("error out"=w344:errorcluster, "Histogram Report"=w360:T20)  [unwired: 9 in]
              n111 = Unbundle By Name(w360) -> ("Mean Value"=w361:sgl)
              n112 = call "IMAQ Convolute"("Kernel"=w364, "Image Dst"=w355, "Image Src"=w358) -> ("error out"=w351:errorcluster)  [unwired: 7 in, 1 out]
              n113 = Multiply(x=w361, y="Blink Sensitivity") -> (x*y=w362:sgl)
              n114 = call "IMAQ Convolute"("Kernel"=w363, "Image Dst"=w354, "Image Src"=w358) -> ("error out"=w350:errorcluster)  [unwired: 7 in, 1 out]
              n115 = call "IMAQ Compare"("Constant"=w362, "Operator"=T13."Clear  if < ", "error in (no error)"=w344, "Image Dst"=w357, "Image Src A"=w353) -> ("error out"=w349:errorcluster)  [unwired: 5 in, 1 out]
              n116 = Merge Errors(w351, w350, w349) -> (w348:errorcluster)
              n117 = Select(t=SMS_Image_Preview_Actions."Exit Loop", s=w348, f=SMS_Image_Preview_Actions."Subtract > Dilate" ("y")) -> (s? t:f=w346:T7)
            }
            frame "Subtract > Dilate" {
              # "Subtracted Image > Dilated Image"
              # "Subtracted"
              # "Dilated Image"
              n118 = Unbundle By Name(w384) -> ("Conv 5 x 5 (SGL)"=w383:T9, "Subtracted (SGL)"=w382:T9, "Conv 11 x 11 (SGL)"=w381:T9, "Dilated (SGL)"=w378:T9, "Ones 7 x 7"=w379:i32[][], "Subtracted > Dilated (SGL)"=w374:T9)
              n119 = call "IMAQ Subtract"("Image Src A"=w383, "Image Dst"=w382, "Image Src B"=w381) -> ("Image Dst Out"=w375:T9, "error out"=w372:errorcluster)  [unwired: 4 in]
              n120 = call "IMAQ GrayMorphology"("Structuring Element"=w379, "error in (no error)"=w372, "Operation"=T14."Dilate", "Image Dst"=w378, "Image Src"=w375) -> ("error out"=w371:errorcluster, "Image Dst Out"=w376:T9)  [unwired: 5 in]
              n121 = call "IMAQ Compare"("Operator"=T13."Clear  if < ", "error in (no error)"=w371, "Image Src B"=w376, "Image Dst"=w374, "Image Src A"=w375) -> ("error out"=w370:errorcluster)  [unwired: 5 in, 1 out]
              n122 = Select(t=SMS_Image_Preview_Actions."Exit Loop", s=w370, f=SMS_Image_Preview_Actions."And Image" ("y")) -> (s? t:f=w367:T7)
            }
            frame "And Image" {
              n123 = Unbundle By Name(w396) -> ("Subtracted > Dilated (SGL)"=w395:T9, "Subtracted > Dilated (U16)"=w394:T9, "And Image (U16)"=w393:T9, "Threshold (U16)"=w392:T9)
              n124 = case shown="\"1\"" enum16{"0", "1"}."1" {
                tunnel: w395 -> [w404 w414]
                tunnel: w394 -> [w403 w413]
                tunnel: w393 -> [w401 w408]
                tunnel: w392 -> [w400 _]
                tunnel: [w398 w409] -> w388
                frame "0" {
                  w405 = T2 7 items=["Grayscale (U8)", "Grayscale (I16)", "Grayscale (SGL)", "Complex (CSG)", "RGB (U32)", "HSL (U32)", "RGB (U64)", "Grayscale (U16)"] ("Image Type")
                  # "Convert to 16 bit for AND operator."
                  # "Does not perform AND operation on \"single\" data type images."
                  n125 = call "IMAQ Cast Image"("Image Type"=w405, "Image Dst"=w403, "Image Src"=w404) -> ("error out"=w399:errorcluster, "Image Dst Out"=w402:T9)  [unwired: 7 in]
                  n126 = call "IMAQ And"("And/Nand (And)"=FALSE, "error in (no error)"=w399, "Image Src B"=w400, "Image Dst"=w401, "Image Src A"=w402) -> ("error out"=w398:errorcluster)  [unwired: 5 in, 1 out]
                }
                frame "1" {
                  w410 = T2 7 items=["Grayscale (U8)", "Grayscale (I16)", "Grayscale (SGL)", "Complex (CSG)", "RGB (U32)", "HSL (U32)", "RGB (U64)", "Grayscale (U16)"] ("Image Type")
                  n127 = call "IMAQ Cast Image"("Image Type"=w410, "Image Dst"=w413, "Image Src"=w414) -> ("error out"=w411:errorcluster, "Image Dst Out"=w412:T9)  [unwired: 7 in]
                  n128 = local read "Blink Sensitivity"() -> (w415:sgl)
                  n129 = call "IMAQ Compare"("Constant"=w415, "Operator"=T13."Clear  if < ", "error in (no error)"=w411, "Image Dst"=w408, "Image Src A"=w412) -> ("error out"=w409:errorcluster, "Image Dst Out"=w407:T9)  [unwired: 5 in]
                  n130 = call "IMAQ Divide"("Image Src A"=w407, "Image Dst"=w408, "Image Src B"=w407) -> ()  [unwired: 4 in, 2 out]
                }
              }
              n131 = Select(t=SMS_Image_Preview_Actions."Exit Loop", s=w388, f=SMS_Image_Preview_Actions."Remove Edge" ("y")) -> (s? t:f=w387:T7)
            }
            frame "Remove Edge" {
              n132 = Unbundle By Name(w432) -> ("Edge Removed (U16)"=w431:T9, "And Image (U16)"=w441:T9, "SMS Preview (U16)"=w419:T9)
              n133 = call "IMAQ ImageToArray"("Image"=w441) -> ("Image Pixels (U16)"=w433:u16[][], "error out"=w428:errorcluster)  [unwired: 3 in, 3 out]
              n134 = Array Size(array=w433) -> (size(s)=w434:i32[])
              n135 = Index Array(array=w434, index #1=0 ("index"), index #2=1 ("index")) -> (element #1=w438:i32, element #2=w439:i32)
              n136 = Multiply(x="Edge Size", y=2) -> (x*y=w422:i32)
              n137 = Subtract(x=w438, y=w422) -> (x-y=w437:i32)
              n138 = Subtract(x=w439, y=w422) -> (x-y=w436:i32)
              n139 = Array Subset(array=w433, index (row)="Edge Size", length (row)=w437, index (col)="Edge Size", length (col)=w436) -> (w430:u16[][])
              n140 = call "IMAQ ArrayToImage"("Image Pixels (U16)"=w430, "error in (no error)"=w428, "Image"=w431) -> ("error out"=w421:errorcluster, "Image Out"=w420:T9)  [unwired: 7 in]
              n141 = case shown="False" "Accumulate" {
                tunnel: w420 -> [w446 w449]
                tunnel: w419 -> [w445 w450]
                tunnel: w421 -> [w444 w448]
                tunnel: [w443 w447] -> w418
                frame False {
                  n142 = call "IMAQ Copy"("error in (no error)"=w444, "Image Dst"=w445, "Image Src"=w446) -> ("error out"=w443:errorcluster)  [unwired: 3 in, 1 out]
                }
                frame True {
                  n143 = call "IMAQ Add"("Image Src A"=w450, "Image Src B"=w449, "error in (no error)"=w448) -> ("error out"=w447:errorcluster)  [unwired: 4 in, 1 out]
                }
              }
              n144 = Select(t=SMS_Image_Preview_Actions."Exit Loop", s=w418, f=SMS_Image_Preview_Actions."Update Plot" ("y")) -> (s? t:f=w424:T7)
            }
            frame "Update Plot" {
              n145 = Unbundle By Name(w467) -> ("Edge Removed (U16)"=w461:T9)
              n146 = call "IMAQ DLL - Num Not Zero.vi"("IMAQ Ref"=w461) -> ("Non Zero Px Total"=w463:u16, "Error Out"=w466:errorcluster)  [unwired: 12 in, 1 out]
              n147 = while {
                tunnel: w463 -> [w476]
                shift-right: [w475] -> w460
                shift-left: _ -> [w474]
                tunnel: "Average Frame No." -> [w472]
                stop <- TRUE ("stop") stop-if-true
                n148 = Array Size(array=w474) -> (size(s)=w471:i32)
                n149 = Greater?(x=w471, y=w472) -> (0:w473:bool)
                n150 = case shown="True" w473 {
                  tunnel: w476 -> [w482 w488]
                  tunnel: [w481 w487] -> w475
                  tunnel: w474 -> [w485 w486]
                  tunnel: w472 -> [w480 _]
                  tunnel: w471 -> [w479 _]
                  frame True {
                    n151 = Subtract(x=w479, y=w480) -> (x-y=w478:i32)
                    n152 = Delete From Array(array=w485, length=w478, index=0) -> (array with subset deleted=w483:u16[])  [unwired: 1 out]
                    n153 = Build Array (concatenate)(w483, w482) -> (w481:u16[])
                  }
                  frame False {
                    n154 = Build Array (concatenate)(w486, w488) -> (w487:u16[])
                  }
                }
              }
              n155 = To Double Precision Float(number=w460) -> (double precision float=w459:dbl[])
              n156 = call-poly <vilib>:"Mean.vi"("X"=w459) -> ("mean"=w458:dbl)  [unwired: 1 out]
              n157 = local read "Lock Density"() -> (w456:bool)
              n158 = case shown="False" "Reset Plot" {
                tunnel: [enum16{"Read", "Write", "Reset"}."Write" ("Plot Data Actions") enum16{"Read", "Write", "Reset"}."Reset" ("Plot Data Actions")] -> w465
                frame False {
                }
                frame True {
                }
              }
              n159 = To Unsigned Word Integer(number=w458) -> (unsigned 16bit integer=w451:u16)
              "Current Emitter No." <- w451
              n160 = Select(t=SMS_Image_Preview_Actions."Update Duration", s=w456, f=SMS_Image_Preview_Actions."Abort" ("y")) -> (s? t:f=w453:T7)
              n161 = call "SMS Image Preview Plot Data.vi"("Plot Data Actions"=w465, "Blink Number"=w451) -> ("Plot Data"=→"Blink No. vs. Time":cluster{dbl[], u16[]})  [unwired: 13 in]
              n162 = Select(t=SMS_Image_Preview_Actions."Exit Loop" ("y"), s=w466, f=w453) -> (s? t:f=w469:T7)
            }
            frame "Update Duration" {
              n163 = Unbundle By Name(w508) -> ("FPGA Notifier Name"=w516:string)
              n164 = local read "Current Emitter No."() -> (w498:u16)
              n165 = To Double Precision Float(number="Target Emitter No.") -> (double precision float=w492:dbl)
              n166 = To Double Precision Float(number=w498) -> (double precision float=w497:dbl)
              n167 = case shown="0, Default" 0 {
                tunnel: [1.0 w520] -> w495
                tunnel: w492 -> [_ w520]
                frame 0, Default {
                }
                frame 1 {
                }
              }
              n168 = Subtract(x=w492, y=w497) -> (x-y=w496:dbl)
              n169 = Divide(x=w496, y=w495) -> (x/y=w518:dbl)
              n170 = Multiply(x=w518, y="P Const.") -> (x*y=w494:dbl)
              n171 = To Double Precision Float(number="Duration") -> (double precision float=w503:dbl)
              n172 = Add(x=w503, y=w494) -> (x+y=w506:dbl)
              n173 = In Range and Coerce(upper limit=0.0, x=w506, lower limit=65535.0) -> (coerced(x)=w500:dbl)  [unwired: 1 out]
              n174 = local read "Laser"() -> (w491:u16)
              n175 = To Unsigned Long Integer(number=w500) -> (unsigned 32bit integer=w499:u32)
              n176 = call "FPGA Messenger.vi"("FPGA Action"=FPGA_Action."Set Duration" ("Action"), "Duration"=w499, "Laser Channel"=w491, "Notifier Name"=w516) -> ("Duration"=w507:u32, "Write Confirm"=w512:bool)  [unwired: 2 in, 4 out]
              n177 = local write "Duration"(w507) -> ()
              n178 = Select(t=SMS_Image_Preview_Actions."Abort" ("y"), s=w512, f=SMS_Image_Preview_Actions."Exit Loop") -> (s? t:f=w510:T7)
            }
            frame "Abort" {
              n179 = Get Notifier Status(notifier=w530) -> (current notification=w529:T8)  [unwired: 1 in, 4 out]
              n180 = Unbundle By Name(w529) -> ("Action"=w528:T7)
              n181 = Equal?(x=SMS_Image_Preview_Actions."Abort" ("y"), y=w528) -> (x = y?=w525:bool)
              n182 = local read "Use Quadrant"() -> (w522:bool)
              n183 = case shown="True" w522 {
                tunnel: [SMS_Image_Preview_Actions."Get Image" ("f") SMS_Image_Preview_Actions."Get Quad" ("f")] -> w521
                frame False {
                }
                frame True {
                }
              }
              n184 = Select(t=SMS_Image_Preview_Actions."Exit Loop", s=w525, f=w521) -> (s? t:f=w526:T7)
            }
            frame "Exit Loop" {
              n185 = local write "Duration"(u32 0 ("Duration")) -> ()
            }
            frame "Quit" {
              n186 = Release Notifier(notifier=w551) -> (last notification=w550:T8)  [unwired: 2 in, 2 out]
              n187 = Unbundle By Name(w550) -> ("SMS Preview (U16)"=w549:T9, "Camera ROI (U16)"=w547:T9, "Threshold (U16)"=w546:T9, "Subtracted > Dilated (U16)"=w545:T9, "And Image (U16)"=w544:T9, "Camera ROI (SGL)"=w543:T9, "Conv 5 x 5 (SGL)"=w542:T9, "Conv 11 x 11 (SGL)"=w541:T9, "Subtracted (SGL)"=w540:T9, "Dilated (SGL)"=w539:T9, "Subtracted > Dilated (SGL)"=w538:T9)
              n188 = Build Array(w549, w547, w546, w545, w544, w543, w542, w541, w540, w539, w538) -> (w548:T9[])
              n189 = for {
                tunnel: w548 -> [w555] mode=indexing
                n190 = call "IMAQ Dispose"("Image"=w555) -> ()  [unwired: 5 in, 1 out]
              }
            }
          }
        }
      }
      n191 = while {
        tunnel: w161 -> [w559]
        tunnel: w159 -> [w558]
        tunnel: [FALSE] -> w160
        tunnel: w157 -> [w556]
        stop <- w560 stop-if-true
        n192 = event shown="[6] \"SMS Preview\": Value Change" {
          selector: _ -> [_ _ _ _ _ _ _ _ _]
          dyn-events: _ -> [_ _ _ _ _ _ _ _ _]
          timeout: -1 -> [_ _ _ _ _ _ _ _ _]
          tunnel: FALSE -> [w563 w567 w581 w588 w612 w636 w670 w680 _]
          tunnel: [w563 w567 w581 w588 w612 w636 w670 w680 w686] -> w560
          tunnel: w559 -> [_ _ w580 _ _ _ _ _ _]
          tunnel: w558 -> [_ _ w578 w587 w596 w639 w669 w679 w685]
          tunnel: w556 -> [_ _ _ _ _ _ _ w674 _]
          event Timeout {
            n193 = event-data() -> ()  [unwired: 1 in, 1 out]
          }
          event Application Instance Close? {
            n194 = event-data() -> ()  [unwired: 1 in, 1 out]
            n195 = control-ref of="This VI"() -> (w564:refnum<vi>)
            n196 = invoke class="VI" method="FP.Open"(reference=w564, "Activate"=TRUE ("Activate?"), "State"=T15."Standard") -> ()  [unwired: 2 in, 5 out]
            n197 = event-data("Discard?"=TRUE) -> ()  [unwired: 1 in, 1 out]
          }
          event "Camera": Value Change {
            # "Empty ROI"
            n198 = event-data() -> ("NewVal"=w579:i32)  [unwired: 1 in]
            n199 = Index Array(array=w580, index=w579) -> (element=w571:string)
            n200 = call "Orca Flash Messanger.vi"("Notifier Name"=w571, "Camera Actions"=Orca_Flash_Actions."STATUS") -> ("Notifier Name Dup"=w573:string, "Image Ref"=w572:T9)  [unwired: 9 in, 3 out]
            n201 = Get Notifier Status(notifier=w578) -> (notifier out=w577:refnum<notifier>, current notification=w576:T8)  [unwired: 1 in, 3 out]
            n202 = Bundle By Name(cluster=w576, "Action"=SMS_Image_Preview_Actions."Idle", "Camera Notifier Name"=w573, "Camera Image (U16)"=w572, "Camera ROI"=T16 {"Global Rectangle"=[], "Contours"=[]}) -> (w575:T8)
            n203 = Send Notification(notification=w575, notifier=w577) -> ()  [unwired: 1 in, 2 out]
          }
          event "Camera ROI": Value Change {
            n204 = event-data() -> ()  [unwired: 1 in, 1 out]
            n205 = Get Notifier Status(notifier=w587) -> (notifier out=w586:refnum<notifier>, current notification=w582:T8)  [unwired: 1 in, 3 out]
            n206 = Unbundle By Name(w582) -> ("Camera Image (U16)"=w585:T9)
            n207 = call "SMS Image Preview Select ROI.vi"("Camera Image Ref"=w585) -> ("Camera ROI"=w583:T16, "Canceled?"=w584:bool)  [unwired: 13 in]
            n208 = case shown="False" w584 {
              tunnel: w586 -> [w594 _]
              tunnel: w583 -> [w592 _]
              tunnel: w582 -> [w593 _]
              frame False {
                n209 = Bundle By Name(cluster=w593, "Camera ROI"=w592, "Action"=SMS_Image_Preview_Actions."Idle") -> (w591:T8)
                n210 = property on="SMS Preview" class="Bool (strict)"("DisabledEnum"=T5."Enabled" ("Disabled")) -> ()  [unwired: 2 in, 2 out]
                n211 = Send Notification(notification=w591, notifier=w594) -> ()  [unwired: 1 in, 2 out]
              }
              frame True {
              }
            }
          }
          event "Image Display": Value Change {
            n212 = event-data() -> ("NewVal"=w595:bool)  [unwired: 1 in]
            n213 = Get Notifier Status(notifier=w596) -> (current notification=w597:T8)  [unwired: 1 in, 4 out]
            n214 = Unbundle By Name(w597) -> ("SMS Preview (U16)"=w611:T9)
            n215 = Obtain Notifier(name (unnamed)="Display Module IMAQ Refs", notification data type=T9[] [], create if not found? (T)=FALSE) -> (notifier out=w604:refnum<notifier>, error out=w605:errorcluster)  [unwired: 1 in, 1 out]
            n216 = Get Notifier Status(notifier=w604, error in (no error)=w605) -> (notifier out=w603:refnum<notifier>, current notification=w601:T9[], error out=w602:errorcluster)  [unwired: 2 out]
            n217 = case shown="True" w595 {
              tunnel: w603 -> [w620 w633]
              tunnel: w602 -> [w614 w632]
              tunnel: w601 -> [w616 w631]
              tunnel: [w615 w628] -> w598
              tunnel: [w620 w633] -> w600
              tunnel: [w614 w632] -> w599
              tunnel: w611 -> [w613 w630]
              frame False {
                n218 = Equal?(x=w616, y=w613) -> (x = y?=w619:bool[])
                n219 = for {
                  tunnel: w619 -> [w627] mode=indexing
                  tunnel: [w626] -> w617
                  i -> [w626]
                  stop <- w627 stop-if-true
                }
                n220 = Or Array Elements(Boolean array=w619) -> (logical OR=w618:bool)
                n221 = case shown="False" w618 {
                  tunnel: w617 -> [_ w624]
                  tunnel: w616 -> [w621 w623]
                  tunnel: [w621 w622] -> w615
                  frame False {
                  }
                  frame True {
                    n222 = Delete From Array(array=w623, length=1, index=w624) -> (array with subset deleted=w622:T9[])  [unwired: 1 out]
                  }
                }
              }
              frame True {
                n223 = Insert Into Array(array=w631, index=0, new element=w630) -> (w628:T9[])
              }
            }
            n224 = Send Notification(notification=w598, notifier=w600, error in (no error)=w599) -> (notifier out=w606:refnum<notifier>, error out=w607:errorcluster)
            n225 = Release Notifier(notifier=w606, error in (no error)=w607) -> ()  [unwired: 1 in, 3 out]
          }
          event "Lock Density": Value Change {
            n226 = event-data() -> ("NewVal"=w635:bool)  [unwired: 1 in]
            n227 = Get Notifier Status(notifier=w639) -> (current notification=w634:T8)  [unwired: 1 in, 4 out]
            n228 = Unbundle By Name(w634) -> ("Laser Notifier Name"=w638:string, "FPGA Notifier Name"=w637:string)
            n229 = case shown="True" w635 {
              tunnel: w638 -> [_ w661]
              tunnel: w637 -> [w640 w659]
              frame False {
                w641 = u16 0 items=["Off", "On", "Rising", "Falling", "Camera"] ("Laser Mode")
                n230 = call "FPGA Messenger.vi"("FPGA Action"=FPGA_Action."Set Laser Mode" ("Action"), "Laser Mode"=w641, "Laser Channel"=u16 0, "Notifier Name"=w640) -> ()  [unwired: 2 in, 6 out]
              }
              frame True {
                w658 = u16 2 items=["Off", "On", "Rising", "Falling", "Camera"] ("Laser Mode")
                n231 = local read "Laser"() -> (w644:u16)
                n232 = Bundle By Name(cluster=T18 {"Laser Parameters"=enum."Wavelength (nm)", "Value"=0.0} ("Settings"), "Laser Parameters"=Laser_Parameters."External Control", "Value"=1.0) -> (w645:T18)
                n233 = call "FPGA Messenger.vi"("FPGA Action"=FPGA_Action."Set Laser Mode" ("Action"), "Laser Mode"=w658, "Laser Channel"=w644, "Notifier Name"=w659) -> ("Laser Channel"=w654:u16, "Notifier Name Out"=w657:string)  [unwired: 2 in, 4 out]
                n234 = call "FPGA Messenger.vi"("Sequence"=fxp<+,16,16> 65535.0, "FPGA Action"=FPGA_Action."Set Sequence" ("Action"), "Laser Channel"=w654, "Notifier Name"=w657) -> ("Laser Channel"=w653:u16, "Notifier Name Out"=w655:string)  [unwired: 2 in, 4 out]
                n235 = local read "Duration"() -> (w649:u32)
                n236 = call "Laser Messenger.vi"("Notifier Name"=w661, "Action"=Laser_Actions."Set Parameter", "Laser Settings"=w645) -> ()  [unwired: 7 in, 6 out]
                n237 = call "FPGA Messenger.vi"("FPGA Action"=FPGA_Action."Set Duration" ("Action"), "Duration"=w649, "Laser Channel"=w653, "Notifier Name"=w655) -> ()  [unwired: 2 in, 6 out]
              }
            }
          }
          event "SMS Preview": Value Change {
            n238 = event-data() -> ("NewVal"=w665:bool)  [unwired: 1 in]
            n239 = Get Notifier Status(notifier=w669) -> (notifier out=w668:refnum<notifier>, current notification=w667:T8)  [unwired: 1 in, 3 out]
            n240 = Select(t=SMS_Image_Preview_Actions."Start SMS Preview" ("Action"), s=w665, f=SMS_Image_Preview_Actions."Abort") -> (s? t:f=w662:T7)
            n241 = Bundle By Name(cluster=w667, "Action"=w662) -> (w666:T8)
            n242 = Send Notification(notification=w666, notifier=w668) -> ()  [unwired: 1 in, 2 out]
          }
          event "Laser": Value Change {
            n243 = event-data() -> ("NewVal"=w673:u16)  [unwired: 1 in]
            n244 = Get Notifier Status(notifier=w679) -> (notifier out=w678:refnum<notifier>, current notification=w677:T8)  [unwired: 1 in, 3 out]
            n245 = Index Array(array=w674, index=w673) -> (element=w672:string)
            n246 = Bundle By Name(cluster=w677, "Action"=SMS_Image_Preview_Actions."Idle", "Laser Notifier Name"=w672) -> (w676:T8)
            n247 = Send Notification(notification=w676, notifier=w678) -> ()  [unwired: 1 in, 2 out]
            n248 = local write "Lock Density"(FALSE ("Lock Density")) -> ()
          }
          event "Quit": Value Change {
            n249 = event-data() -> ("NewVal"=w686:bool)  [unwired: 1 in]
            n250 = Get Notifier Status(notifier=w685) -> (notifier out=w683:refnum<notifier>, current notification=w682:T8)  [unwired: 1 in, 3 out]
            n251 = Bundle By Name(cluster=w682, "Action"=SMS_Image_Preview_Actions."Quit") -> (w684:T8)
            n252 = Send Notification(notification=w684, notifier=w683) -> ()  [unwired: 1 in, 2 out]
          }
        }
      }
      n253 = local write "Quit"(w160) -> ()
    }
  }
  n254 = property class="Pnl"(reference=w98) -> ("Decos[]"=w96:refnum<vi>[], "Panes[]"=w102:refnum<vi>[])  [unwired: 1 in, 2 out]
  n255 = Array Size(array=w96) -> (size(s)=w94:i32)
  n256 = Decrement(x=w94) -> (x-1=w95:i32)
  n257 = Index Array(array=w102, index=0) -> (element=w101:refnum<vi>)
  n258 = Index Array(array=w96, index=w95) -> (element=w104:refnum<vi>)
  n259 = property class="VI"(reference=w106) -> (reference out=w108:refnum<vi>, "Front Panel.PanelBounds"=w109:T21)  [unwired: 1 in, 1 out]
  n260 = property class="Decor"(reference=w104) -> ("Bounds"=w107:T22)  [unwired: 1 in, 2 out]
  n261 = property class="Pane"(reference=w101, "Origin"=T11 {"Horizontal"=0, "Vertical"=0}, "HorizScrollbarVisibility"=w105, "VertScrollbarVisibility"=w105) -> ()  [unwired: 1 in, 2 out]
  n262 = Unbundle By Name(w107) -> ("Width"=w112:u32, "Height"=w115:u32)
  n263 = control-ref of="Quit"() -> (w99:refnum<vi>)
  n264 = To Word Integer(number=w112) -> (16bit integer=w114:i16)
  n265 = To Word Integer(number=w115) -> ()  [unwired: 1 out]
  n266 = property class="Bool (strict)"(reference=w99) -> ("Height"=w117:u32, "Top"=w118:i32)  [unwired: 1 in, 2 out]
  n267 = Unbundle By Name(w109) -> ("Left"=w111:i16, "Top"=w122:i16)
  n268 = To Word Integer(number=w117) -> (16bit integer=w120:i16)
  n269 = To Word Integer(number=w118) -> (16bit integer=w121:i16)
  n270 = Add(x=w111, y=w114) -> (x+y=w113:i16)
  n271 = Compound Arithmetic op=ADD(w122, w120, w121, i16 12 ("y")) -> (w116:i16)
  n272 = Bundle By Name(cluster=w109, "Right"=w113, "Bottom"=w116) -> (w110:T21)
  n273 = property class="VI"(reference=w108, "Front Panel.PanelBounds"=w110) -> ()  [unwired: 1 in, 2 out]
